vi "File Name of Python Module--constant.vi"() -> (3 "File Name of Python Module":string)   [LabVIEW 2026]
doc: "This constant defines the name of the productively used python module in the generated project."
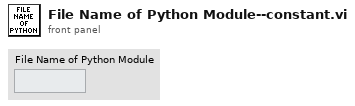
[diagram p1: front panel]
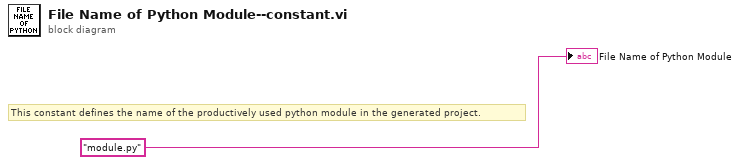
[diagram p0: block diagram]
diagram:
  # "This constant defines the name of the productively used python module in the generated project."
  "File Name of Python Module" <- "module.py" ("File Name of Python Module")
